vi "Update Account Balance.vi"(8 "error in":errorcluster, 9 "New Balance":dbl, 10 "Account Number":string, 11 "Accounts File Path":path) -> (0 "error out":errorcluster)   [LabVIEW 2026]
doc: "Sets the balance of one account in the ATM accounts file (read-modify-write). All records are read with Read Accounts.vi, the account is located with Find Account.vi, only its Balance is replaced, and the whole file is written back in the same CSV format (Account Number,First Name,Last Name,Balance; one record per line, LF line endings). Balance is written with a period as decimal separator and without trailing zeros (550 -> 550, 1000.5 -> 1000.5). If the account is not in the file, error 5002 is returned and the file is left untouched. The file reference is always closed."
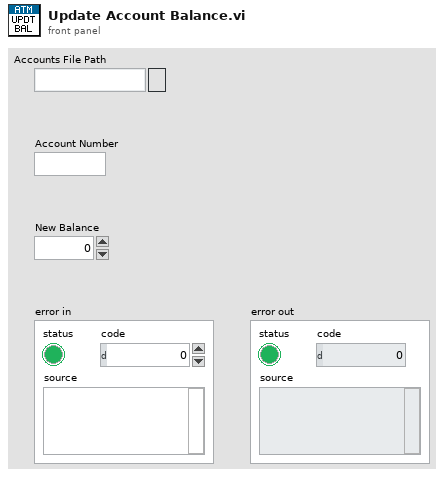
[diagram p1: front panel]
types:
  T1 = typedef "ATM Account.ctl" = cluster{"Account Number":string, "First Name":string, "Last Name":string, "Balance":dbl}
  T2 = enum16{"open", "replace", "create", "open or create", "replace or create", "replace or create with confirmation"}
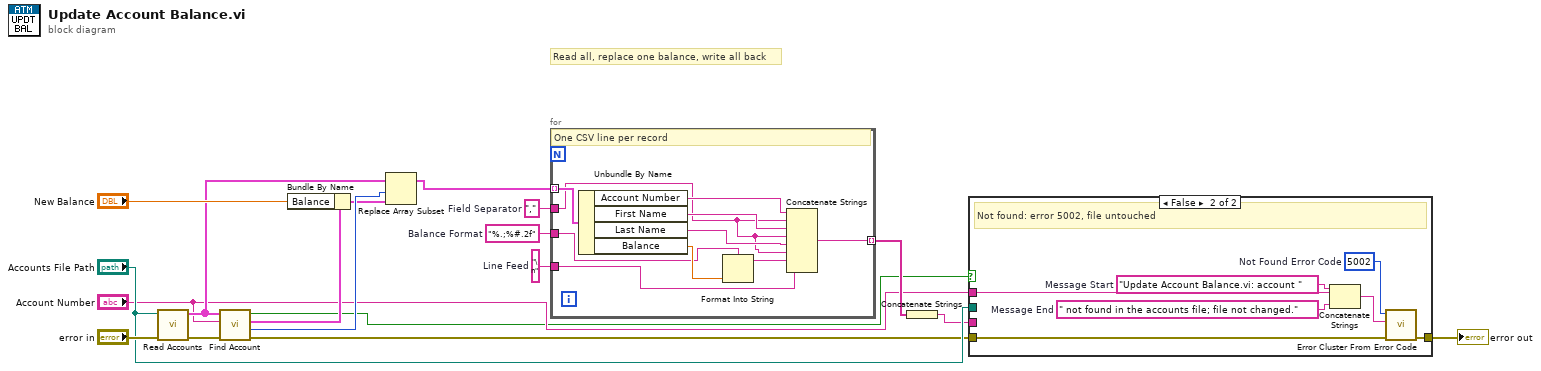
[diagram p0: block diagram]
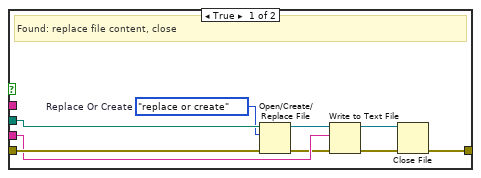
[diagram p2: hidden frame]
diagram:
  w8 = "\n"  # Line Feed
  w9 = ","  # Field Separator
  w10 = "%.;%#.2f"  # Balance Format
  # "Read all, replace one balance, write all back"
  n1 = call "Read Accounts.vi"("error in"="error in", "Accounts File Path"="Accounts File Path") -> ("error out"=w17:errorcluster, "Accounts"=w14:T1[])  [unwired: 8 in]
  n2 = call "Find Account.vi"("error in"=w17, "Account Number"="Account Number", "Accounts"=w14) -> ("error out"=w4:errorcluster, "Index"=w13:i32, "Account"=w15:T1, "Account Found?"=w2:bool)  [unwired: 5 in]
  n3 = Bundle By Name(cluster=w15, "Balance"="New Balance") -> (w12:T1)
  n4 = Replace Array Subset(array=w14, new element=w12, index=w13) -> (w11:T1[])
  n5 = for {
    tunnel: w11 -> [w28] mode=indexing
    tunnel: w10 -> [w26]
    tunnel: w9 -> [w22]
    tunnel: w8 -> [w20]
    tunnel: [w19] -> w7 mode=indexing
    # "One CSV line per record"
    n6 = Unbundle By Name(w28) -> ("Account Number"=w25:string, "First Name"=w24:string, "Last Name"=w23:string, "Balance"=w27:dbl)
    n7 = Format Into String(format string=w26, w27) -> (resulting string=w21:string)  [unwired: 2 in, 1 out]
    n8 = Concatenate Strings(w25, w22, w24, w22, w23, w22, w21, w20) -> (w19:string)
  }
  n9 = Concatenate Strings(w7) -> (w5:string)
  n10 = case shown="False" w2 {
    tunnel: "Accounts File Path" -> [w37 _]
    tunnel: w5 -> [w33 _]
    tunnel: w4 -> [w35 w40]
    tunnel: "Account Number" -> [_ w43]
    tunnel: [w29 w38] -> w1
    frame True {
      w36 = T2."replace or create"  # Replace Or Create
      # "Found: replace file content, close"
      n11 = Open/Create/Replace File(file path (use dialog)=w37, error in=w35, operation (0:open)=w36) -> (refnum out=w34:refnum<file>, error out=w32:errorcluster)  [unwired: 3 in, 1 out]
      n12 = Write to Text File(file (use dialog)=w34, text=w33, error in=w32) -> (refnum out=w31:refnum<file>, error out=w30:errorcluster)  [unwired: 1 in, 1 out]
      n13 = Close File(refnum=w31, error in=w30) -> (error out=w29:errorcluster)  [unwired: 1 out]
    }
    frame False {
      w42 = " not found in the accounts file; file not changed."  # Message End
      w44 = "Update Account Balance.vi: account "  # Message Start
      w41 = 5002  # Not Found Error Code
      # "Not found: error 5002, file untouched"
      n14 = Concatenate Strings(w44, w43, w42) -> (w39:string)
      n15 = call <vilib>:"Error Cluster From Error Code.vi"("error in (no error)"=w40, "error message (\"\")"=w39, "error code (0)"=w41) -> ("error out"=w38:errorcluster)  [unwired: 6 in]
    }
  }
  "error out" <- w1
